vi "Volts_to_pa.vi"(2 "P_max_Pa":dbl=103421.0, 3 "P_min_Pa":dbl, 4 "V_supply":dbl=5.13, 5 "V_in":dbl) -> (0 "P_Pa":dbl, 1 "Out_of_range":bool)   [LabVIEW 2025]
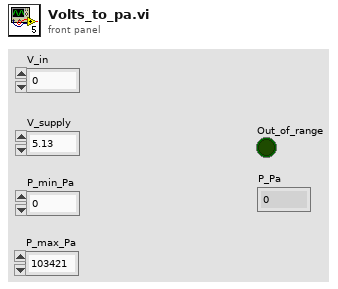
[diagram p1: front panel]
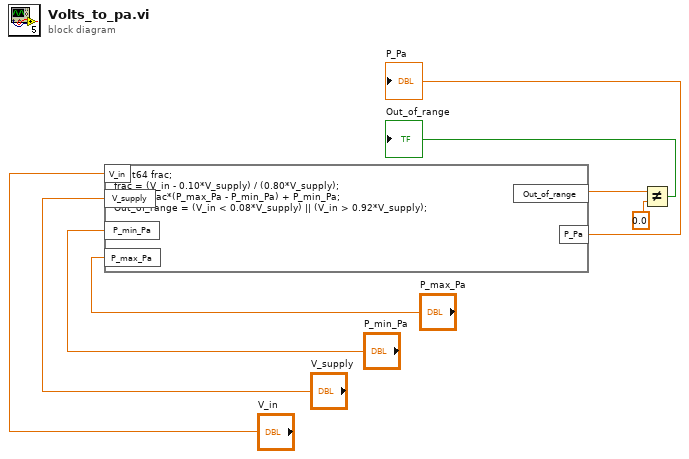
[diagram p0: block diagram]
diagram:
  n1 = formula code="float64 frac;\nfrac = (V_in - 0.10*V_supply) / (0.80*V_supply);\nP_Pa = frac*(P_max_Pa - P_min_Pa) + P_min_Pa;\nOut_of_range = (V_in < 0.08*V_supply) || (V_in > 0.92*V_supply);"("P_min_Pa"="P_min_Pa", "P_max_Pa"="P_max_Pa", "V_in"="V_in", "V_supply"="V_supply") -> ("P_Pa"=→"P_Pa":dbl, "Out_of_range"=w3:dbl)
  n2 = Not Equal?(x=w3, y=0.0) -> (x != y?=→"Out_of_range":bool)
